vi "drugie.vi"() -> ()   [LabVIEW 2026]
uses:
  <vilib>/Analysis/3filter.llb/Filter Passband Type.ctl
  <vilib>/ptbypt/NI_PtbyPt.lvlib
  <vilib>/Analysis/NI_AALBase.lvlib
panel:
  in  "stop":bool
  in  "Czêstotliwoœæ graniczna filtra [Hz]":dbl(slide) scale=0.1..1.0
  in  "okres próbkowania [s]":dbl(slide) scale=0.0..4.0
  out "Waveform Chart":cluster{"Biezaca_dana":dbl, "Filtered x":dbl}(graph)
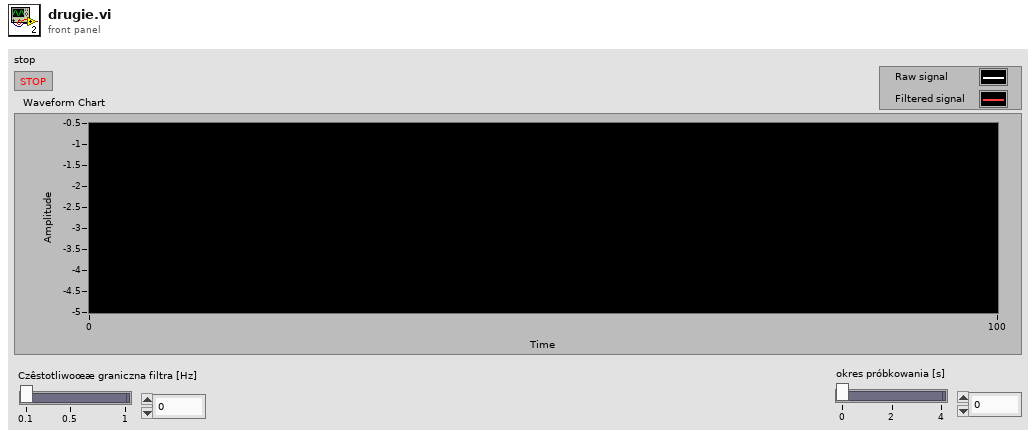
[diagram p1: front panel]
types:
  T1 = typedef "NI_AALBase.lvlib/Filter Passband Type.ctl" = enum32{"Lowpass", "Highpass", "Bandpass", "Bandstop"}
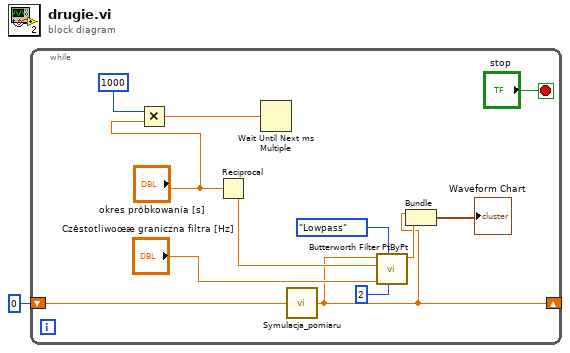
[diagram p0: block diagram]
diagram:
  n1 = while {
    shift-right: [w5] -> _
    shift-left: 0 -> [w13]
    stop <- "stop" stop-if-true
    n2 = Multiply(x=1000, y="okres próbkowania [s]") -> (x*y=w2:dbl)
    n3 = Reciprocal(x="okres próbkowania [s]") -> (1/x=w8:dbl)
    n4 = Wait Until Next ms Multiple(millisecond multiple=w2) -> ()  [unwired: 1 out]
    n5 = call "Symulacja_pomiaru.vi"("poprzednia_dana"=w13) -> ("Biezaca_dana"=w5:dbl)
    n6 = call <vilib>:"Butterworth Filter PtByPt.vi"("order"=2, "filter type"=Filter_Passband_Type."Lowpass", "low cutoff freq: fl"="Czêstotliwoœæ graniczna filtra [Hz]", "sampling freq: fs"=w8, "x"=w5) -> ("Filtered x"=w6:dbl)  [unwired: 4 in, 1 out]
    n7 = Bundle("Biezaca_dana"=w5, "Filtered x"=w6) -> (→"Waveform Chart":cluster{"Biezaca_dana":dbl, "Filtered x":dbl})  [unwired: 1 in]
  }
